vi "Stop Core.vi"(10 "final error code":i32, 11 "CommonState in":refnum<class "CoordinatorState.lvclass">) -> (3 "CommonState out":refnum<class "CoordinatorState.lvclass">)   [LabVIEW 2014, in "States.lvlib" / "CoordinatorState.lvclass"]
doc: "(<B>Filename</B>: Actor Framework.lvlib:Actor.lvclass:Stop Core.vi)\n\nThis override stops the nested Process Actor.\n\nDefines what the actor does before it stops. Use the <B>final error code</B> input to determine whether the actor shut down in response to an error.\n\nBy default, this method does nothing. A descendant class may override it to define behavior, such as shutting down any processes the actor initiated in its override of the Actor Core method."
uses:
  CoordinatorState.lvclass
  <vilib>/ActorFramework/Actor/Actor.lvclass/Actor.ctl
  CoordinatorState.lvclass/CoordinatorState.ctl
  <vilib>/ActorFramework/Stop Msg/Stop Msg.lvclass/Stop Msg.ctl
  <vilib>/ActorFramework/Message Enqueuer/Message Enqueuer.lvclass/Message Enqueuer.ctl
  <vilib>/ActorFramework/Stop Msg/Send Emergency Stop.vi
  <vilib>/ActorFramework/Stop Msg/Send Normal Stop.vi
  <vilib>/ActorFramework/Message Enqueuer/Enqueue Critical.vi
  <vilib>/ActorFramework/Message Enqueuer/Enqueue.vi
  <vilib>/ActorFramework/Message Priority Queue/Priority Enqueue.vi
  <vilib>/NI/Actors/State Actor/State Actor/State Actor.lvclass
  <vilib>/ActorFramework/Stop Msg/Stop Msg.lvclass
  <vilib>/ActorFramework/Actor/Actor.lvclass
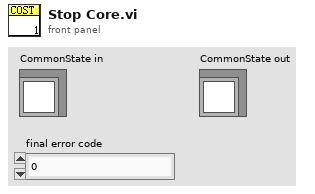
[diagram p1: front panel]
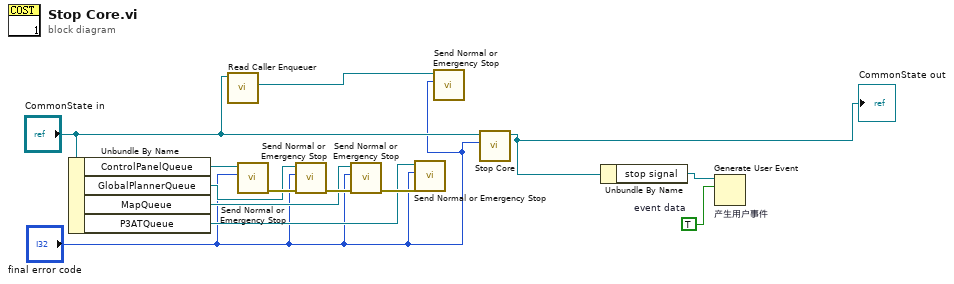
[diagram p0: block diagram]
diagram:
  w11 = TRUE  # event data
  n1 = Unbundle By Name("CommonState in") -> ("ControlPanelQueue"=w13:refnum<class "Message Enqueuer.lvclass">, "GlobalPlannerQueue"=w8:refnum<class "Message Enqueuer.lvclass">, "MapQueue"=w6:refnum<class "Message Enqueuer.lvclass">, "P3ATQueue"=w4:refnum<class "Message Enqueuer.lvclass">)
  n2 = call <vilib>:"Read Caller Enqueuer.vi"("Actor"="CommonState in") -> ("Caller Enqueuer"=w1:refnum<class "Message Enqueuer.lvclass">)  [unwired: 10 in]
  n3 = call <vilib>:"Send Normal or Emergency Stop.vi"("final error code"="final error code", "Message Enqueuer"=w13) -> ("error out"=w9:errorcluster)  [unwired: 9 in]
  n4 = call <vilib>:"Send Normal or Emergency Stop.vi"("error in (no error)"=w9, "final error code"="final error code", "Message Enqueuer"=w8) -> ("error out"=w7:errorcluster)  [unwired: 8 in]
  n5 = call <vilib>:"Send Normal or Emergency Stop.vi"("error in (no error)"=w7, "final error code"="final error code", "Message Enqueuer"=w6) -> ("error out"=w5:errorcluster)  [unwired: 8 in]
  n6 = call <vilib>:"Send Normal or Emergency Stop.vi"("error in (no error)"=w5, "final error code"="final error code", "Message Enqueuer"=w4) -> ()  [unwired: 8 in, 1 out]
  n7 = call <vilib>:"Send Normal or Emergency Stop.vi"("final error code"="final error code", "Message Enqueuer"=w1) -> ()  [unwired: 9 in, 1 out]
  n8 = call-parent "Stop Core.vi"("final error code"="final error code", "Actor in"="CommonState in") -> ("Actor out"=w10:refnum<class "CoordinatorState.lvclass">)  [unwired: 9 in]
  "CommonState out" <- w10
  n9 = Unbundle By Name(w10) -> ("stop signal"=w12:refnum<user-event>)
  n10 = Generate User Event "产生用户事件"(user event=w12, event data cluster=w11) -> ()  [unwired: 2 in, 2 out]
